vi "Exp - Get CalcExpress Error as Error Cluster.vi"(7 "InstanceRef":T1, 8 "error in":errorcluster, 11 "Get CE Error (T)":bool=TRUE) -> (0 "error out":errorcluster, 3 "dup Get CE Error":bool=TRUE)   [LabVIEW 2021]
doc: "Use this VI to retrieve a CalcExpress error as the standard LabVIEW error cluster. Refer to the VI help for more details.\n\nThis VI runs normally if <b>error in</b> does not indicate any error. If <b>Get CE Error</b> is TRUE (default), the VI calls the CalcExpress Engine to retrieve the error information. If an error occurred prior to the execution of this VI, information on that error is returned in the <b>error out</b> cluster.\n\nMost FuncVI support VIs use Boolean <b>error in</b> and <b>error out</b>. You can wire <b>Get CE Error</b> to the Boolean <b>error out</b> indicator of these VIs for data flow.\n\n::: CalcExpress Toolkit :::\nCopyright (c) 2000-2026 Konstantin Shifershteyn. All rights reserved."
uses:
  cetypes.llb/CalcExpress Instance RefNum.ctl
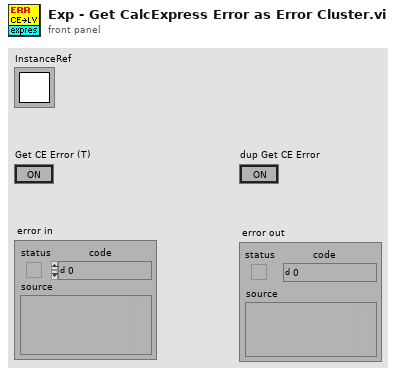
[diagram p1: front panel]
types:
  T1 = typedef "CalcExpress Instance RefNum.ctl" = refnum<k1>
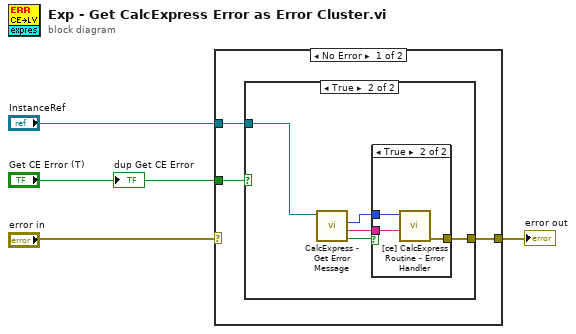
[diagram p0: block diagram]
diagram:
  n1 = case shown="No Error" "error in" {
    selector: "error in" -> [_ w16]
    tunnel: "InstanceRef" -> [w7 _]
    tunnel: "Get CE Error (T)" -> [w6 _]
    tunnel: [w5 w16] -> w2
    frame No Error {
      n2 = case shown="True" w6 {
        tunnel: w7 -> [_ w9]
        tunnel: [_ w12] -> w5
        frame False {
        }
        frame True {
          n3 = call "CalcExpress - Get Error Message.vi"("CE InstanceRef"=w9) -> ("error out"=w8:bool, "error description"=w10:string, "error code"=w11:i32)  [unwired: 5 in, 1 out]
          n4 = case shown="True" w8 {
            tunnel: w11 -> [_ w15]
            tunnel: w10 -> [_ w14]
            tunnel: [_ w13] -> w12
            frame False {
            }
            frame True {
              n5 = call "[ce] CalcExpress Routine - Error Handler.vi"("error msg"=w14, "error code"=w15) -> ("error out"=w13:errorcluster)  [unwired: 7 in]
            }
          }
        }
      }
    }
    frame Error {
    }
  }
  "error out" <- w2
  "dup Get CE Error" <- "Get CE Error (T)"
